vi "get_sine_point__6cd72d9aa1.vi"(7 "relative seconds":dbl, 8 "Initial position in voltage":dbl, 9 "voltage to displacement constant":dbl, 10 "amplitude":dbl=1.0 format="%0.2f", 11 "frequency":dbl=1.0 format="%0.2f") -> (1 "resulting string":string, 2 "Elapsedf time (s)":dbl, 3 "set point":dbl)   [LabVIEW 2023]
uses:
  <vilib>/ptbypt/NI_PtbyPt.lvlib
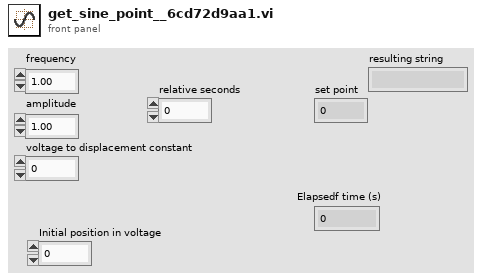
[diagram p1: front panel]
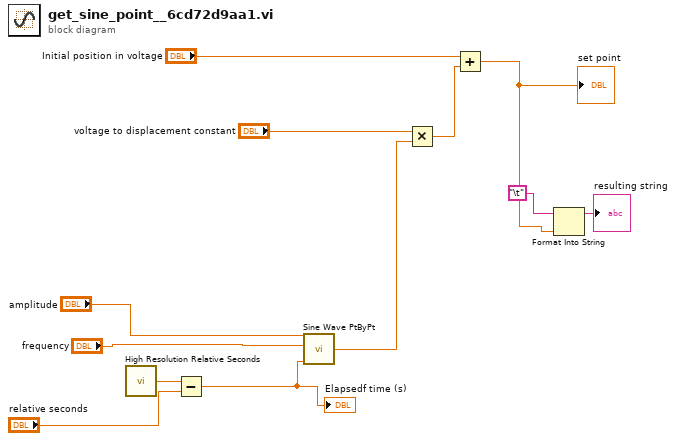
[diagram p0: block diagram]
diagram:
  n1 = call <vilib>:"High Resolution Relative Seconds.vi"() -> ("relative seconds"=w10:dbl)
  n2 = Subtract(x=w10, y="relative seconds") -> (x-y=w12:dbl)
  "Elapsedf time (s)" <- w12
  n3 = call <vilib>:"Sine Wave PtByPt.vi"("time"=w12, "frequency"="frequency", "amplitude"="amplitude") -> ("sine wave"=w6:dbl)  [unwired: 1 in]
  n4 = Multiply(x="voltage to displacement constant", y=w6) -> (x*y=w4:dbl)
  n5 = Add(x="Initial position in voltage", y=w4) -> (x+y=w3:dbl)
  "set point" <- w3
  n6 = Format Into String(initial string="\t", w3) -> (resulting string=→"resulting string":string)  [unwired: 2 in, 1 out]
